vi "AeroTray_Control_Formula.vi"() -> ()   [LabVIEW 2019]
uses:
  <vilib>/myRIO/Instrument Drivers/Onboard IO/DIO/typedefs/DIO Reference.ctl
  <vilib>/myRIO/Common/Instrument Driver Framework/Utilities/typedefs/myRIO Generic Hardware Reference.ctl
  <vilib>/myRIO/Common/Instrument Driver Framework/Utilities/typedefs/Hardware Version Enum.ctl
  <vilib>/myRIO/Common/Instrument Driver Framework/Utilities/typedefs/myRIO v1.0 Reference.ctl
  <vilib>/myRIO/Common/Instrument Driver Framework/Utilities/typedefs/Generic FPGA Reference.ctl
  <vilib>/myRIO/Common/Instrument Driver Framework/myRIO v1.0/DIO/typedefs/DIO Channels List.ctl
  <vilib>/myRIO/Common/Instrument Driver Framework/myRIO v1.0/DIO/typedefs/DIO Channels Enum.ctl
  <vilib>/userDefined/High Color/nirio_resource_hc.ctl
  <vilib>/myRIO/Instrument Drivers/Onboard IO/PWM/typedefs/PWM Reference.ctl
  <vilib>/myRIO/Common/Instrument Driver Framework/myRIO v1.0/PWM/typedefs/PWM Channels Enum.ctl
  <vilib>/myRIO/Instrument Drivers/Onboard IO/PWM/typedefs/PWM Configuration.ctl
  <vilib>/myRIO/Common/Instrument Driver Framework/myRIO v1.0/DIO/vis/myRIO v1.1 Open DIO.vi
  <vilib>/myRIO/Common/Instrument Driver Framework/myRIO v1.0/PWM/vis/myRIO v1.1 Open PWM.vi
  <vilib>/myRIO/Common/Instrument Driver Framework/Utilities/vis/Validate Channels.vi
  <vilib>/myRIO/Common/Instrument Driver Framework/myRIO v1.0/DIO/vis/myRIO v1.0 Reserve DIO.vi
  <vilib>/myRIO/Common/Instrument Driver Framework/myRIO v1.0/PWM/vis/myRIO v1.0 Reserve PWM.vi
  <vilib>/myRIO/Instrument Drivers/Onboard IO/PWM/vis/Set Duty Cycle and Frequency.vi
  <vilib>/myRIO/Common/Instrument Driver Framework/myRIO v1.0/DIO/vis/myRIO v1.0 Close DIO.vi
  <vilib>/myRIO/Common/Instrument Driver Framework/myRIO v1.0/PWM/vis/myRIO v1.0 Close PWM.vi
  <vilib>/myRIO/Common/Instrument Driver Framework/myRIO v1.0/Resource Manager/vis/myRIO v1.0 Reserve Channel List.vi
  <vilib>/myRIO/Common/Instrument Driver Framework/myRIO v1.0/DIO/vis/myRIO v1.0 Build MUX Configuration DIO.vi
  <vilib>/myRIO/Common/Instrument Driver Framework/myRIO v1.0/PWM/vis/myRIO v1.0 Build MUX Configuration PWM.vi
  <vilib>/myRIO/Common/Instrument Driver Framework/myRIO v1.0/DIO/vis/myRIO v1.0 Unreserve DIO.vi
  <vilib>/myRIO/Common/Instrument Driver Framework/myRIO v1.0/PWM/vis/myRIO v1.0 Unreserve PWM.vi
  <vilib>/myRIO/Common/Instrument Driver Framework/myRIO v1.0/Resource Manager/vis/myRIO v1.0 Reserve Channel.vi
  <vilib>/myRIO/Common/Instrument Driver Framework/myRIO v1.0/Resource Manager/vis/myRIO v1.0 Unreserve Channel.vi
  <vilib>/myRIO/Common/Instrument Driver Framework/myRIO v1.0/Resource Manager/vis/myRIO v1.0 Create Configuration List.vi
  <vilib>/myRIO/Common/Instrument Driver Framework/myRIO v1.0/Resource Manager/vis/myRIO v1.0 Unreserve Channel List.vi
  <vilib>/myRIO/Common/Instrument Driver Framework/myRIO v1.0/Resource Manager/vis/myRIO v1.0 Build Mutex Name.vi
  <vilib>/Utility/VariantDataType/GetNumericInfo.vi
  <vilib>/Utility/error.llb/Error Cluster From Error Code.vi
  <vilib>/myRIO/Common/Instrument Driver Framework/myRIO v1.0/myRIO v1.1 Open.vi
  <vilib>/myRIO/Common/Instrument Driver Framework/Utilities/vis/IO Manager.vi
  <vilib>/myRIO/Common/Instrument Driver Framework/Utilities/vis/Configuration Manager.vi
  <vilib>/myRIO/Common/Instrument Driver Framework/myRIO v1.0/Resource Manager/vis/myRIO v1.0 Configure IO.vi
  <vilib>/myRIO/Common/Instrument Driver Framework/myRIO v1.0/myRIO v1.0 Close.vi
  <vilib>/myRIO/Common/Instrument Driver Framework/myRIO v1.0/PWM/vis/myRIO v1.0 Write PWM.vi
  <vilib>/myRIO/Common/Instrument Driver Framework/myRIO v1.0/DIO/vis/myRIO v1.0 Write DIO.vi
  <vilib>/myRIO/Common/Instrument Driver Framework/myRIO v1.0/DIO/vis/myRIO v1.0 Shutdown DIO.vi
  <vilib>/myRIO/Common/Instrument Driver Framework/myRIO v1.0/PWM/vis/myRIO v1.0 Shutdown PWM.vi
  <vilib>/myRIO/Instrument Drivers/Onboard IO/PWM/vis/myRIO PWM Open.xnode
  <vilib>/myRIO/Instrument Drivers/Onboard IO/DIO/vis/myRIO DIO Open.xnode
  <vilib>/myRIO/Instrument Drivers/Onboard IO/PWM/PWM.lvlib
  <vilib>/myRIO/Instrument Drivers/Onboard IO/DIO/DIO.lvlib
panel:
  out "dir_der":dbl
  out "dir_izq":dbl
  out "pwm_der":dbl
  out "pwm_izq":dbl
  in  "finalizar":dbl
  in  "stop_emergencia":dbl=1.0
  in  "duty_pct":dbl
  in  "comando":dbl
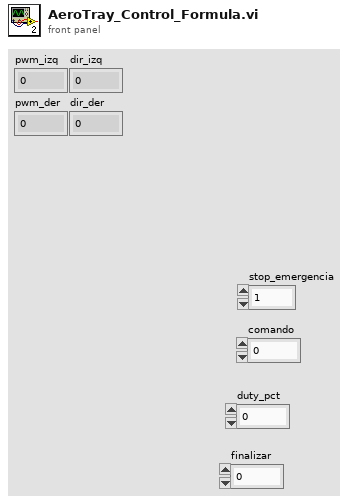
[diagram p1: front panel]
types:
  T1 = typedef "DIO.lvlib/DIO Reference.ctl" = cluster{"myRIO Reference":T2, "DIO Channels List":T6}
  T2 = typedef "myRIO Generic Hardware Reference.ctl" = cluster{"myRIO Model":T3, "myRIO Hardware Reference":T4}
  T3 = typedef "Hardware Version Enum.ctl" = enum16{"Unknown", "myRIO-1900", "myRIO-1950", "roboRIO", "NI ELVIS RIO CM", "ELVIS III"}
  T4 = typedef "myRIO v1.0 Reference.ctl" = cluster{"Generic FPGA Reference":T5, "Allow multiple opens":bool}
  T5 = typedef "Generic FPGA Reference.ctl" = refnum<k20>
  T6 = typedef "DIO Channels List.ctl" = T7[]
  T7 = typedef "DIO Channels Enum.ctl" = enum16{"Not Connected", "C/DIO0", "C/DIO1", "C/DIO2", "C/DIO3", "C/DIO4", "C/DIO5", "C/DIO6", "C/DIO7", "A/DIO0", "A/DIO1", "A/DIO2", "A/DIO3", "A/DIO4", "A/DIO5", "A/DIO6", "A/DIO7", "A/DIO8", "A/DIO9", "A/DIO10", "A/DIO11", "A/DIO12", "A/DIO13", "A/DIO14", "A/DIO15", "A/DIO16", "A/DIO17", "A/DIO18", "A/DIO19", "B/DIO0", "B/DIO1", "B/DIO2", "B/DIO3", "B/DIO4", "B/DIO5", "B/DIO6", "B/DIO7", "B/DIO8", "B/DIO9", "B/DIO10", "B/DIO11", "B/DIO12", "B/DIO13", "B/DIO14", "B/DIO15", "B/DIO16", "B/DIO17", "B/DIO18", "B/DIO19", "LED0", "LED1", "LED2", "LED3", "Button0", "DIO/DIO0", "DIO/DIO1", "DIO/DIO2", "DIO/DIO3", "DIO/DIO4", "DIO/DIO5", "DIO/DIO6", "DIO/DIO7", "DIO/DIO8", "DIO/DIO9", "SPI/CS0", "SPI/CS1", "SPI/CS2", "SPI/CS3", "LED RADIO (Green)", "LED RADIO (Red)", "LED COMM (Green)", "LED COMM (Red)", "LED MODE (Green)", "LED MODE (Red)"}
  T8 = typedef "PWM.lvlib/PWM Reference.ctl" = cluster{"myRIO Reference":T2, "PWM Channels Enum":T9, "PWM Configuration":T10}
  T9 = typedef "PWM Channels Enum.ctl" = enum16{"Not Connected", "C/PWM0", "C/PWM1", "A/PWM0", "A/PWM1", "A/PWM2", "A/PWM3", "A/PWM4", "A/PWM5", "A/PWM6", "A/PWM7", "A/PWM8", "A/PWM9", "A/PWM10", "A/PWM11", "A/PWM12", "A/PWM13", "A/PWM14", "A/PWM15", "A/PWM16", "A/PWM17", "A/PWM18", "A/PWM19", "B/PWM0", "B/PWM1", "B/PWM2", "B/PWM3", "B/PWM4", "B/PWM5", "B/PWM6", "B/PWM7", "B/PWM8", "B/PWM9", "B/PWM10", "B/PWM11", "B/PWM12", "B/PWM13", "B/PWM14", "B/PWM15", "B/PWM16", "B/PWM17", "B/PWM18", "B/PWM19", "PWM/PWM0", "PWM/PWM1", "PWM/PWM2", "PWM/PWM3", "PWM/PWM4", "PWM/PWM5", "PWM/PWM6", "PWM/PWM7", "PWM/PWM8", "PWM/PWM9"}
  T10 = typedef "PWM.lvlib/PWM Configuration.ctl" = cluster{"Frequency":dbl, "Duty Cycle":dbl}
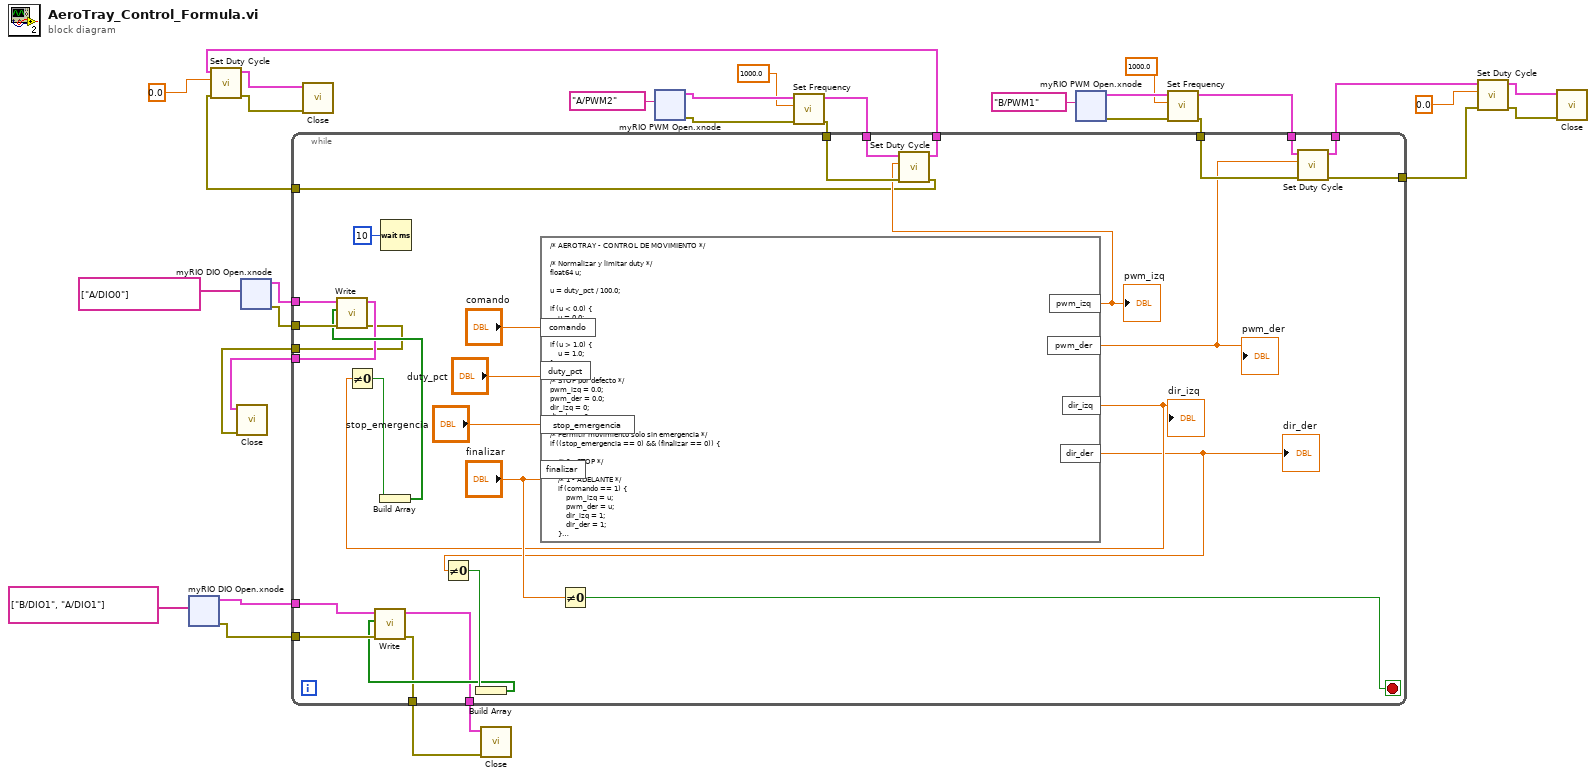
[diagram p0: block diagram]
diagram:
  n1 = xnode "myRIO DIO Open.xnode"("Channel Names"=tag[] ["B/DIO1", "A/DIO1"]) -> ("error out"=w15:errorcluster, "DIO Ref Out"=w16:T1)  [unwired: 2 in]
  n2 = xnode "myRIO DIO Open.xnode"("Channel Names"=tag[] ["A/DIO0"]) -> ("error out"=w24:errorcluster, "DIO Ref Out"=w25:T1)  [unwired: 2 in]
  n3 = xnode "myRIO PWM Open.xnode"("Channel Name"=tag "A/PWM2") -> ("error out"=w32:errorcluster, "PWM Ref Out"=w31:T8)  [unwired: 2 in]
  n4 = call <vilib>:"Set Frequency.vi"("error in (no error)"=w32, "Frequency [Hz]"=1000.0, "PWM Ref In"=w31) -> ("error out"=w27:errorcluster, "PWM Ref Out"=w28:T8)  [unwired: 6 in]
  n5 = xnode "myRIO PWM Open.xnode"("Channel Name"=tag "B/PWM1") -> ("error out"=w20:errorcluster, "PWM Ref Out"=w22:T8)  [unwired: 2 in]
  n6 = call <vilib>:"Set Frequency.vi"("error in (no error)"=w20, "Frequency [Hz]"=1000.0, "PWM Ref In"=w22) -> ("error out"=w18:errorcluster, "PWM Ref Out"=w19:T8)  [unwired: 6 in]
  n7 = while {
    tunnel: w28 -> [w56]
    tunnel: w27 -> [w55]
    tunnel: w25 -> [w53]
    tunnel: w24 -> [w52]
    tunnel: w19 -> [w48]
    tunnel: w18 -> [w47]
    tunnel: w16 -> [w45]
    tunnel: w15 -> [w44]
    tunnel: [w40] -> w13
    tunnel: [w39] -> w12
    tunnel: [w38] -> w8
    tunnel: [w37] -> w7
    tunnel: [w36] -> w4
    tunnel: [w35] -> w3
    tunnel: [w34] -> w2
    tunnel: [w33] -> w1
    stop <- w58 stop-if-true
    n8 = Wait (ms)(milliseconds to wait=u32 10) -> ()  [unwired: 1 out]
    n9 = formula code="/* AEROTRAY - CONTROL DE MOVIMIENTO */\n\n/* Normalizar y limitar duty */\nfloat64 u;\n\nu = duty_pct / 100.0;\n\nif (u < 0.0) {\n    u = 0.0;\n}\n\nif (u > 1.0) {\n    u = 1.0;\n}\n\n/* STOP por defecto */\npwm_izq = 0.0;\npwm_der = 0.0;\ndir_izq = 0;\ndir_der = 0;\n\n/* Permitir movimiento solo sin emergencia */\nif ((stop_emergencia == 0) && (finalizar == 0)) {\n\n    /* 0 - STOP */\n\n    /* 1 - ADELANTE */\n    if (comando == 1) {\n        pwm_izq = u;\n        pwm_der = u;\n        dir_izq = 1;\n        dir_der = 1;\n    }\n\n    /* 2 - ATRAS */\n    else if (comando == 2) {\n        pwm_izq = u;\n        pwm_der = u;\n        dir_izq = 0;\n        dir_der = 0;\n    }\n\n    /* 3 - GIRO IZQUIERDA */\n    else if (comando == 3) {\n        pwm_izq = u;\n        pwm_der = u;\n        dir_izq = 0;\n        dir_der = 1;\n    }\n\n    /* 4 - GIRO DERECHA */\n    else if (comando == 4) {\n        pwm_izq = u;\n        pwm_der = u;\n        dir_izq = 1;\n        dir_der = 0;\n    }\n}"("comando"="comando", "duty_pct"="duty_pct", "stop_emergencia"="stop_emergencia", "finalizar"="finalizar") -> ("pwm_izq"=w54:dbl, "pwm_der"=w46:dbl, "dir_izq"=w51:dbl, "dir_der"=w42:dbl)
    "pwm_izq" <- w54
    "pwm_der" <- w46
    "dir_izq" <- w51
    "dir_der" <- w42
    n10 = Not Equal To 0?(x=w51) -> (x != 0?=w50:bool)
    n11 = Build Array(w50) -> (w49:bool[])
    n12 = call <vilib>:"Write.vi"("error in (no error)"=w52, "Values"=w49, "DIO Ref In"=w53) -> ("error out"=w35:errorcluster, "DIO Ref Out"=w36:T1)  [unwired: 6 in]
    n13 = Not Equal To 0?(x=w42) -> (x != 0?=w43:bool)
    n14 = Build Array(w43) -> (w41:bool[])
    n15 = call <vilib>:"Write.vi"("error in (no error)"=w44, "Values"=w41, "DIO Ref In"=w45) -> ("error out"=w34:errorcluster, "DIO Ref Out"=w33:T1)  [unwired: 6 in]
    n16 = Not Equal To 0?(x="finalizar") -> (x != 0?=w58:bool)
    n17 = call <vilib>:"Set Duty Cycle.vi"("error in (no error)"=w55, "Duty Cycle"=w54, "PWM Ref In"=w56) -> ("error out"=w39:errorcluster, "PWM Ref Out"=w40:T8)  [unwired: 6 in]
    n18 = call <vilib>:"Set Duty Cycle.vi"("error in (no error)"=w47, "Duty Cycle"=w46, "PWM Ref In"=w48) -> ("error out"=w37:errorcluster, "PWM Ref Out"=w38:T8)  [unwired: 6 in]
  }
  n19 = call <vilib>:"Set Duty Cycle.vi"("error in (no error)"=w12, "Duty Cycle"=0.0, "PWM Ref In"=w13) -> ("error out"=w10:errorcluster, "PWM Ref Out"=w11:T8)  [unwired: 6 in]
  n20 = call <vilib>:"Close.vi"("error in (no error)"=w3, "DIO Ref In"=w4) -> ()  [unwired: 9 in, 1 out]
  n21 = call <vilib>:"Close.vi"("error in (no error)"=w10, "PWM Ref In"=w11) -> ()  [unwired: 9 in, 1 out]
  n22 = call <vilib>:"Close.vi"("error in (no error)"=w2, "DIO Ref In"=w1) -> ()  [unwired: 9 in, 1 out]
  n23 = call <vilib>:"Set Duty Cycle.vi"("error in (no error)"=w7, "Duty Cycle"=0.0, "PWM Ref In"=w8) -> ("error out"=w5:errorcluster, "PWM Ref Out"=w6:T8)  [unwired: 6 in]
  n24 = call <vilib>:"Close.vi"("error in (no error)"=w5, "PWM Ref In"=w6) -> ()  [unwired: 9 in, 1 out]
